vi "Concatenate Non-Empty Strings.vi"(6 "String2":string, 7 "Seperator(Carriage Return)":string="\r", 8 "String1":string) -> (2 "Result String":string)   [LabVIEW 2017, in "CSM Shared.lvlib"]
uses:
  CSM Shared.lvlib
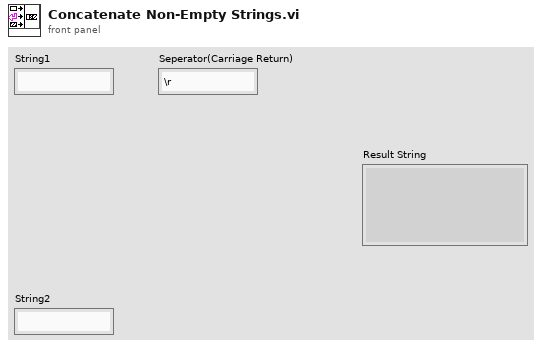
[diagram p1: front panel]
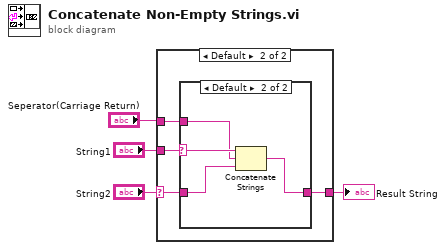
[diagram p0: block diagram]
diagram:
  n1 = case shown="Default" "String2" {
    selector: "String2" -> [_ w8]
    tunnel: [w5 w9] -> w2
    tunnel: "String1" -> [w5 w7]
    tunnel: "Seperator(Carriage Return)" -> [_ w6]
    frame "" {
    }
    frame Default {
      n2 = case shown="Default" w7 {
        selector: w7 -> [_ w13]
        tunnel: [w10 w14] -> w9
        tunnel: w8 -> [w10 w12]
        tunnel: w6 -> [_ w11]
        frame "" {
        }
        frame Default {
          n3 = Concatenate Strings(w13, w11, w12) -> (w14:string)
        }
      }
    }
  }
  "Result String" <- w2
